vi "RemoteVI Route Input.vi"(0 "kind":T3(ring), 1 "panel":T1, 2 "windows":T2(array[cluster]), 3 "key window":u64, 5 "msg":u32, 7 "x":i32, 9 "y":i32, 11 "error in":errorcluster) -> (4 "panel out":T1, 6 "msg out":u32, 8 "key window out":u64, 15 "error out":errorcluster)   [LabVIEW 2020, in "RemoteVI.lvlib"]
doc: "Decides which window one mouse or key message of a client goes to (docs\\protocol.md section 7) and gives the panel cluster RemoteVI Post Client Input.vi then posts with. MOUSE: to the front-most listed window whose client area (x, y, w, h in main-frame coordinates) holds the point - windows is front-most first - else to the panel; while a popup is open, to the window the client last pressed a button in (key window), whose popup it is, else the panel. KEYS: to the front-most modal window, else to key window when it is still listed, else to the panel; inside that window to the child that has the keyboard focus when it belongs to it (RemoteVI Thread Windows.vi + user32 GetAncestor.vi GA_ROOT - the file name box of a native file dialog, where Escape and Enter work like on the host; measured on LabVIEW 2025). For a window the geometry becomes clientX, clientY = its client-area origin on screen (sx, sy); the frame origin stays, because main-frame coordinates are screen offsets. A NATIVE dialog (class #32770) is made of child windows: the point is followed down with user32 ChildWindowFromPointEx.vi to the deepest visible child under it, and the geometry is set so that the posted lParam is that child's CLIENT coordinates in every case (LabVIEW reads screen coordinates while it tracks a press, a Windows control does not). A button-down sets key window out (0 = the panel). While a modal window is listed and no popup is open a mouse message for the panel is dropped (msg out = 0, which RemoteVI Translate Input.vi does not post): LabVIEW would still handle a message posted to its disabled panel, and on the host the panel takes no input then. Win32 calls only, no VI Server."
uses:
  RemoteVI.lvlib
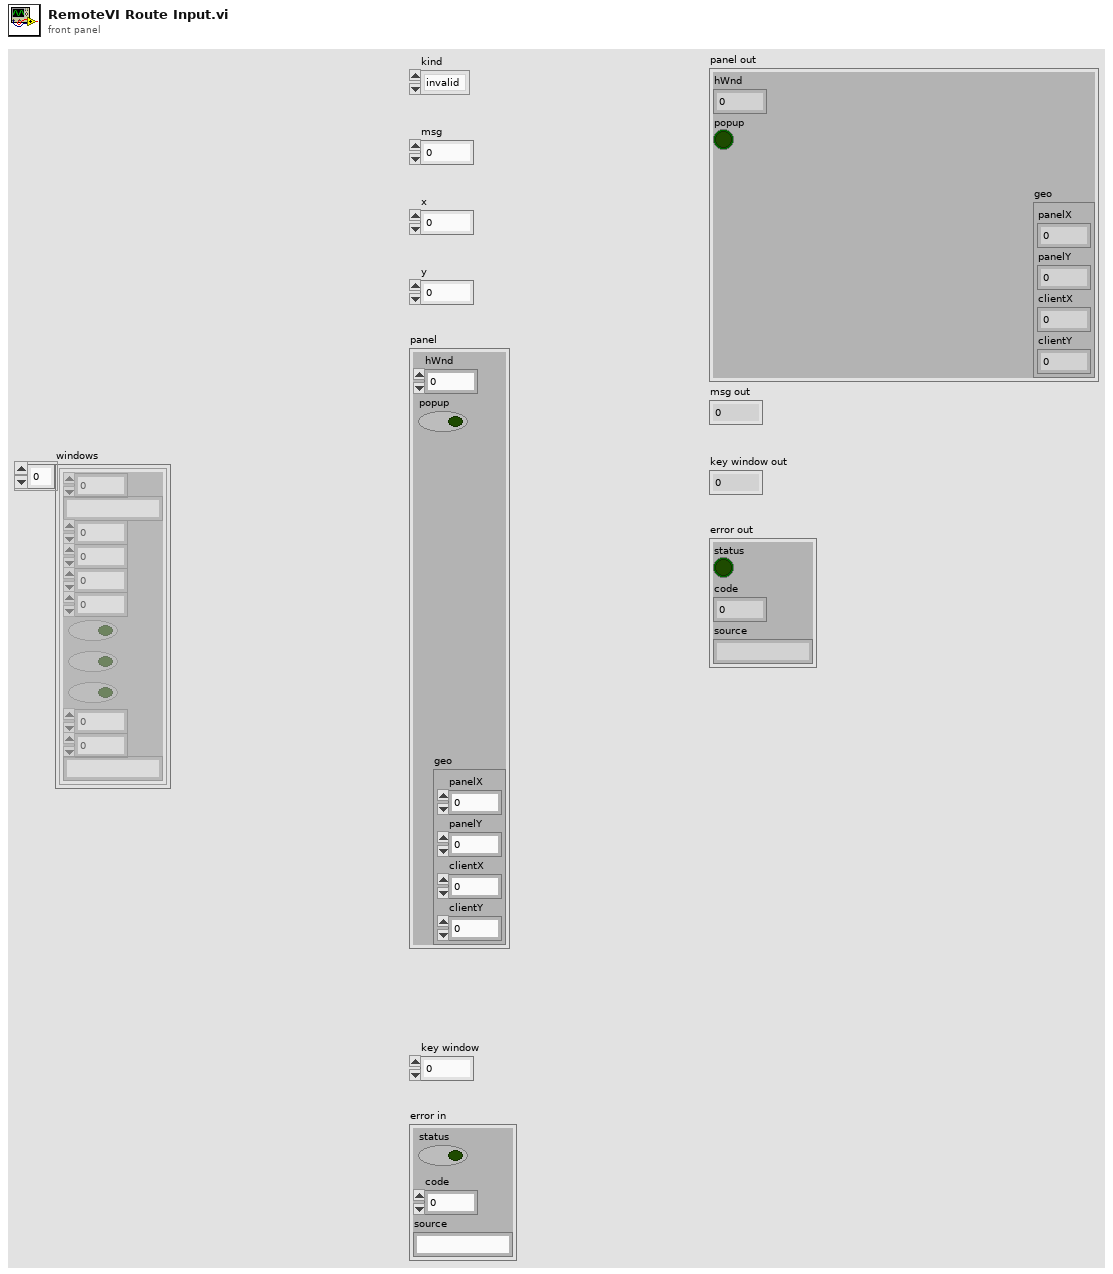
[diagram p1: front panel]
types:
  T1 = cluster{"hWnd":u64, "popup":bool, "geo":cluster{"panelX":i32, "panelY":i32, "clientX":i32, "clientY":i32}}
  T2 = cluster{"id":u64, "title":string, "x":i32, "y":i32, "w":i32, "h":i32, "modal":bool, "active":bool, "closable":bool, "sx":i32, "sy":i32, "class":string}[]
  T3 = enum16{"invalid", "mouse", "key", "ack", "close", "splitter"}
  T4 = cluster{"panelX":i32, "panelY":i32, "clientX":i32, "clientY":i32}
  T5 = cluster{"id":u64, "title":string, "x":i32, "y":i32, "w":i32, "h":i32, "modal":bool, "active":bool, "closable":bool, "sx":i32, "sy":i32, "class":string}
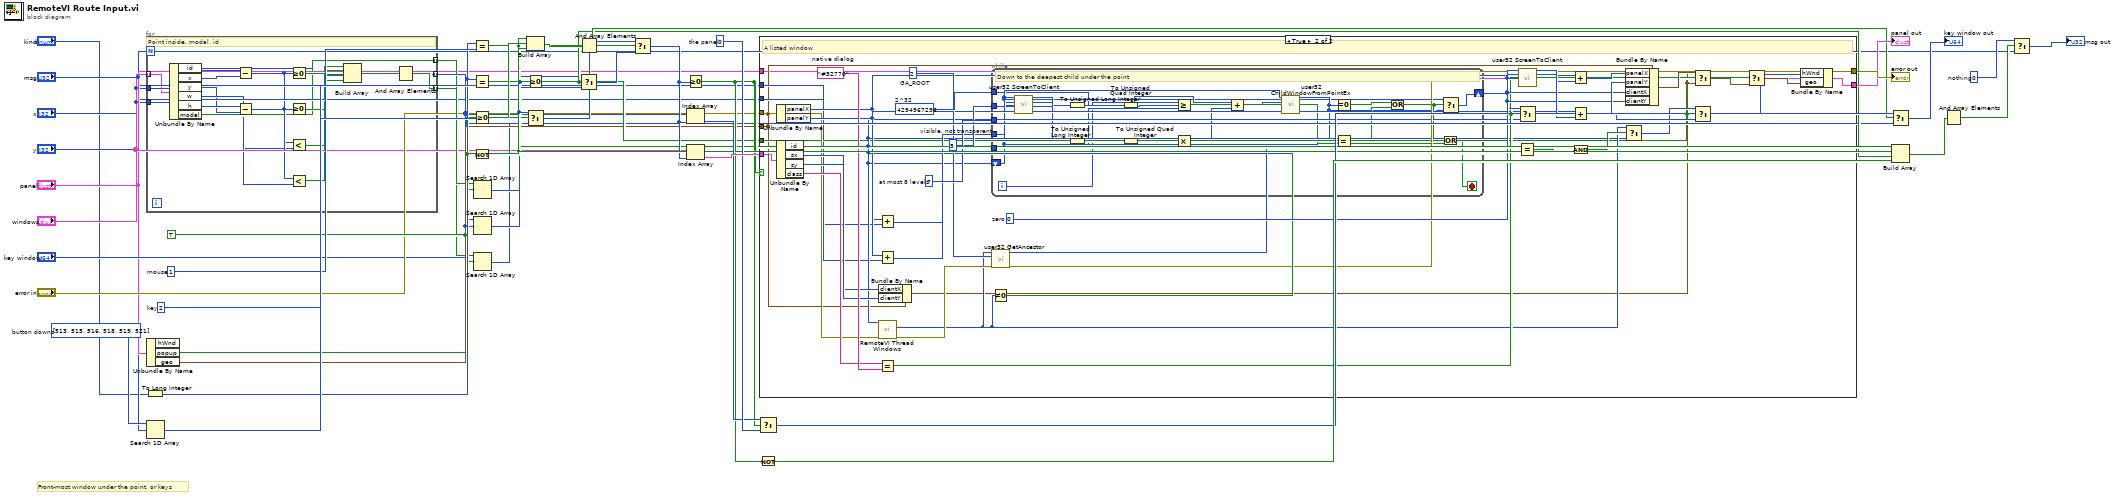
[diagram p0: block diagram]
diagram:
  w41 = u32 0  # nothing
  w35 = u64 0  # the panel
  w28 = u32[] [513, 515, 516, 518, 519, 521]  # button downs
  w21 = 2  # key
  w20 = 1  # mouse
  w12 = TRUE
  # "Front-most window under the point, or keys"
  n1 = for {
    tunnel: "windows" -> [w46] mode=indexing
    tunnel: "x" -> [w47]
    tunnel: "y" -> [w48]
    tunnel: [w54] -> w10 mode=indexing
    tunnel: [w49] -> w11 mode=indexing
    tunnel: [w62] -> w9 mode=indexing
    # "Point inside, modal, id"
    n2 = Unbundle By Name(w46) -> ("id"=w49:u64, "x"=w50:i32, "y"=w51:i32, "w"=w52:i32, "h"=w53:i32, "modal"=w54:bool)
    n3 = Subtract(x=w47, y=w50) -> (x-y=w55:i32)
    n4 = Subtract(x=w48, y=w51) -> (x-y=w56:i32)
    n5 = Greater Or Equal To 0?(x=w55) -> (x >= 0?=w57:bool)
    n6 = Greater Or Equal To 0?(x=w56) -> (x >= 0?=w58:bool)
    n7 = Less?(x=w55, y=w52) -> (x < y?=w59:bool)
    n8 = Less?(x=w56, y=w53) -> (x < y?=w60:bool)
    n9 = Build Array(w57, w58, w59, w60) -> (w61:bool[])
    n10 = And Array Elements(Boolean array=w61) -> (logical AND=w62:bool)
  }
  n11 = Unbundle By Name("panel") -> ("popup"=w17:bool, "geo"=w18:T4)  [unwired: 1 out]
  n12 = To Long Integer(number="kind") -> (32bit integer=w19:i32)
  n13 = Search 1D Array(1D array=w28, element="msg") -> (index of element=w29:i32)  [unwired: 1 in]
  n14 = Equal?(x=w19, y=w20) -> (x = y?=w22:bool)
  n15 = Equal?(x=w19, y=w21) -> (x = y?=w23:bool)
  n16 = Greater Or Equal To 0?(x=w29) -> (x >= 0?=w30:bool)
  n17 = Not(x=w17) -> (.not. x?=w31:bool)
  n18 = Search 1D Array(1D array=w10, element=w12) -> (index of element=w14:i32)  [unwired: 1 in]
  n19 = Search 1D Array(1D array=w11, element="key window") -> (index of element=w15:i32)  [unwired: 1 in]
  n20 = Search 1D Array(1D array=w9, element=w12) -> (index of element=w13:i32)  [unwired: 1 in]
  n21 = Build Array(w22, w30, w31) -> (w32:bool[])
  n22 = Greater Or Equal To 0?(x=w14) -> (x >= 0?=w16:bool)
  n23 = Select(t=w15, s=w17, f=w13) -> (s? t:f=w24:i32)
  n24 = And Array Elements(Boolean array=w32) -> (logical AND=w33:bool)
  n25 = Select(t=w14, s=w16, f=w15) -> (s? t:f=w25:i32)
  n26 = Select(t=w24, s=w22, f=w25) -> (s? t:f=w26:i32)
  n27 = Greater Or Equal To 0?(x=w26) -> (x >= 0?=w27:bool)
  n28 = Index Array(array=w11, index=w26) -> (element=w34:u64)
  n29 = Index Array(array="windows", index=w26) -> (element=w43:T5)
  n30 = case shown="True" w27 {
    tunnel: "panel" -> [w63 w65]
    tunnel: "x" -> [_ w68]
    tunnel: "y" -> [_ w69]
    tunnel: "error in" -> [w64 w71]
    tunnel: w18 -> [_ w67]
    tunnel: w23 -> [_ w70]
    tunnel: w43 -> [_ w66]
    tunnel: [w64 w83] -> w45
    tunnel: [w63 w106] -> w44
    frame False {
      # "The panel"
    }
    frame True {
      w96 = 0  # zero
      w94 = 7  # at most 8 levels
      w93 = u32 5  # visible, not transparent
      w92 = u64 4294967296  # 2^32
      w88 = "#32770"  # native dialog
      w81 = u32 2  # GA_ROOT
      # "A listed window"
      n31 = Unbundle By Name(w67) -> ("panelX"=w76:i32, "panelY"=w77:i32)
      n32 = Unbundle By Name(w66) -> ("id"=w72:u64, "sx"=w73:i32, "sy"=w74:i32, "class"=w75:string)
      n33 = Add(x=w76, y=w68) -> (x+y=w90:i32)
      n34 = Add(x=w77, y=w69) -> (x+y=w91:i32)
      n35 = Bundle By Name(cluster=w67, "clientX"=w73, "clientY"=w74) -> (w78:T4)
      n36 = call "RemoteVI Thread Windows.vi"("hWnd"=w72, "error in"=w71) -> ("focus"=w79:u64, "error out"=w80:errorcluster)  [unwired: 10 in, 2 out]
      n37 = Equal?(x=w75, y=w88) -> (x = y?=w89:bool)
      n38 = while {
        tunnel: w92 -> [w110]
        tunnel: w93 -> [w111]
        tunnel: w94 -> [w112]
        tunnel: w90 -> [w108]
        tunnel: w91 -> [w109]
        shift-right: [w114] -> w95
        shift-left: w72 -> [w113]
        i -> [w107]
        stop <- w128 stop-if-true
        # "Down to the deepest child under the point"
        n39 = call "user32 ScreenToClient.vi"("hWnd"=w113, "Screen X"=w108, "Screen Y"=w109) -> ("Client X"=w115:i32, "Client Y"=w116:i32)  [unwired: 9 in, 2 out]
        n40 = To Unsigned Long Integer(number=w115) -> (unsigned 32bit integer=w117:u32)
        n41 = To Unsigned Long Integer(number=w116) -> (unsigned 32bit integer=w118:u32)
        n42 = To Unsigned Quad Integer(1:w117) -> (0:w119:u64)
        n43 = To Unsigned Quad Integer(1:w118) -> (0:w120:u64)
        n44 = Greater Or Equal?(x=w107, y=w112) -> (x >= y?=w127:bool)
        n45 = Multiply(x=w120, y=w110) -> (x*y=w121:u64)
        n46 = Add(x=w119, y=w121) -> (x+y=w122:u64)
        n47 = call "user32 ChildWindowFromPointEx.vi"("hwnd"=w113, "pt"=w122, "flags"=w111) -> ("child"=w123:u64)  [unwired: 11 in, 1 out]
        n48 = Equal To 0?(x=w123) -> (x = 0?=w124:bool)
        n49 = Equal?(x=w123, y=w113) -> (x = y?=w125:bool)
        n50 = Or(x=w124, y=w125) -> (x .or. y?=w126:bool)
        n51 = Select(t=w113, s=w126, f=w123) -> (s? t:f=w114:u64)
        n52 = Or(x=w126, y=w127) -> (x .or. y?=w128:bool)
      }
      n53 = call "user32 GetAncestor.vi"("hwnd"=w79, "gaFlags"=w81, "error in"=w80) -> ("ancestor"=w82:u64, "error out"=w83:errorcluster)  [unwired: 11 in]
      n54 = Not Equal To 0?(x=w79) -> (x != 0?=w85:bool)
      n55 = call "user32 ScreenToClient.vi"("hWnd"=w95, "Screen X"=w96, "Screen Y"=w96) -> ("Client X"=w97:i32, "Client Y"=w98:i32)  [unwired: 9 in, 2 out]
      n56 = Select(t=w95, s=w89, f=w72) -> (s? t:f=w102:u64)
      n57 = Equal?(x=w82, y=w72) -> (x = y?=w84:bool)
      n58 = Add(x=w76, y=w97) -> (x+y=w99:i32)
      n59 = Add(x=w77, y=w98) -> (x+y=w100:i32)
      n60 = And(x=w84, y=w85) -> (x .and. y?=w86:bool)
      n61 = Bundle By Name(cluster=w67, "panelX"=w99, "panelY"=w100, "clientX"=w96, "clientY"=w96) -> (w101:T4)
      n62 = Select(t=w79, s=w86, f=w72) -> (s? t:f=w87:u64)
      n63 = Select(t=w101, s=w89, f=w78) -> (s? t:f=w103:T4)
      n64 = Select(t=w87, s=w70, f=w102) -> (s? t:f=w104:u64)
      n65 = Select(t=w78, s=w70, f=w103) -> (s? t:f=w105:T4)
      n66 = Bundle By Name(cluster=w65, "hWnd"=w104, "geo"=w105) -> (w106:T1)
    }
  }
  "panel out" <- w44
  "error out" <- w45
  n67 = Select(t=w34, s=w27, f=w35) -> (s? t:f=w36:u64)
  n68 = Not(x=w27) -> (.not. x?=w38:bool)
  n69 = Select(t=w36, s=w33, f="key window") -> (s? t:f=→"key window out":u64)
  n70 = Build Array(w22, w31, w16, w38) -> (w39:bool[])
  n71 = And Array Elements(Boolean array=w39) -> (logical AND=w40:bool)
  n72 = Select(t=w41, s=w40, f="msg") -> (s? t:f=→"msg out":u32)
